vi "MainVI_v1.vi"() -> ()   [LabVIEW 2019]
uses:
  ModBusValue.ctl
  <vilib>/numeric/Random Number (Range) U64.vi
  <vilib>/numeric/sub_Random U32.vi
panel:
  out "문자열[]":string[](array[string])
  in  "아이템 이름":string[][](array[string])=[["1", "Pick&Place Robot", "산업용로봇", "두산로보틱스", "M1509", "ModBusTCP/IP", "192.168.0.100", "200", "대기"], ["2", "", "", "", "", "", "", "", ""], ["3", "", "", "", "", "", "", "", ""], ["4", "", "", "", "", "", "", "", ""], ["5", "", "", "", "", "", "", "", ""], ["6", "", "", "", "", "", "", "", ""], ["7", "", "", "", "", "", "", "", ""], ["8", "", "", "", "", "", "", "", ""], ["9", "", "", "", "", "", "", "", ""], ["10", "", "", "", "", "", "", "", ""], ["11", "", "", "", "", "", "", "", ""]]
  out "Temperature(cobot)":T1
  out "날짜/시간 문자열":string
  out "SystemDataCluster":T2={"문자열 42"="연결", "문자열 43"="연결", "문자열 44"="끊김", "문자열 45"="끊김", "문자열 46"="끊김", "문자열 47"="끊김", "문자열 48"="끊김", "문자열 49"="끊김"} caption="클러스터"
  in  "MAIN Tab":T3(tab)
  out "Cobot_State":string="정지"
  in  "여러 열 리스트박스 4":i32(listbox)
  out "품질률":u8(slide) scale=0.0..100.0
  out "성능률":u8(slide) scale=0.0..100.0
  out "가동률":u8(slide) scale=0.0..100.0
  out "사이클 횟수 그래프":u8(slide) scale=0.0..100.0
  out "웨이브폼 차트 3":u64(graph)=86
  out "AGV_Battery":u8(slide) scale=0.0..100.0
  out "AGV_Coord":string="팔레타이징"
  out "AGV_Action":string="주행 중"
  out "AGV_Velo":string="0.0m"
  out "AGV_UpTime":string="0h00m"
  in  "AGV 통신 리셋":bool
  in  "AGV 통신 정지":bool
  in  "AGV 통신 시작":bool
  out "AGV_State":string="경고"
  out "웨이브폼 차트 2":u64(graph)=86
  out "숫자형 6":dbl
  out "숫자형 7":dbl
  out "숫자형 8":dbl
  out "숫자형 9":dbl
  out "숫자형 5":dbl
  out "숫자형 4":dbl
  out "숫자형 3":dbl
  out "슬라이드 9":u8(slide) scale=0.0..100.0
  out "슬라이드 8":u8(slide) scale=0.0..100.0
  out "슬라이드 7":u8(slide) scale=0.0..100.0
  out "슬라이드 6":u8(slide) scale=0.0..100.0
  out "슬라이드 5":u8(slide) scale=0.0..100.0
  out "슬라이드 4":u8(slide) scale=0.0..100.0
  out "슬라이드 3":u8(slide) scale=0.0..100.0
  out "Cobot_Servo":string="서보 OFF"
  out "Cobot_Task":string="STOP"
  out "Cobot_Cycle":string="0"
  out "Cobot_Comple":string="0/200"
  out "Cobot_UpTime":string="0h00m"
  in  "협동로봇 통신 시작":bool
  in  "협동로봇 통신 리셋":bool
  in  "협동로봇 통신 정지":bool
  out "AMR_Battery":u8(slide) scale=0.0..100.0
  out "AMR_Coord":string="충전스테이션"
  out "AMR_Action":string="주행 중"
  out "AMR_Velo":string="0.0m/s"
  out "AMR_UpTime":string="0h00m"
  in  "AMR 통신 리셋":bool
  in  "AMR 통신 정지":bool
  in  "AMR 통신 시작":bool
  out "AMR_State":string="운전"
  out "Delta_Task":string="자동 검사"
  out "Delta_Cycle":string="0"
  out "Delta_Defective":string="0"
  out "Delta_UpTime":string="0h00m"
  out "Delta_Accuracy":u8(slide) scale=0.0..100.0
  out "IndustRobot_1_Servo":string="서보 OFF"
  out "IndustRobot_1_Task":string="자동 운전"
  out "IndustRobot_1_Cycle":string="100"
  out "IndusRobot_1_Comple":string
  out "IndustRobot_1_UpTime":string="0h00m"
  out "IndustRobot_2_Servo":string="서보 OFF"
  out "IndustRobot_2_Task":string="STOP"
  out "IndustRobot_2_Cycle":string="0"
  out "IndustRobot_2_Comple":string="0"
  out "IndustRobot_2_UpTime":string="0h00m"
  out "IndustRobot_3_Servo":string="서보 OFF"
  out "IndustRobot_3_Task":string="비상 정지"
  out "IndustRobot_3_Cycle":string="0"
  out "IndustRobot_3_Comple":string="0"
  out "IndustRobot_3_UpTime":string="0h00m"
  in  "델타로봇 통신 시작":bool
  in  "델타로봇 통신 리셋":bool
  in  "델타로봇 통신 정지":bool
  in  "산업용로봇 통신 시작":bool
  in  "산업용로봇 통신 리셋":bool
  in  "산업용로봇 통신 정지":bool
  in  "산업용로봇2 통신 시작":bool
  in  "산업용로봇2 통신 리셋":bool
  in  "산업용로봇2 통신 정지":bool
  in  "산업용로봇3 통신 시작":bool
  in  "산업용로봇3 통신 리셋":bool
  in  "산업용로봇3 통신 정지":bool
  out "Delta_State":string="정지"
  out "IndustRobot_1_State":string="정지"
  out "IndustRobot_2_State":string="정지"
  out "IndustRobot_3_State":string="정지"
  out "생산 추이(실시간)":u64(graph)
  out "웨이브폼 차트":u64(graph)=86
  in  "Robot Monitoring Tab":T4(tab)
  in  "Cobot Position Tab":enum32{"Joint Position", "Task Position"}(tab)
  out "Joint Position Graph(cobot)":T5(graph)
  out "Task Position Graph(cobot)":T5(graph)
  in  "여러 열 리스트박스 2":i32(listbox)
  out "Joint6 current":dbl
  out "Joint6 torque":dbl
  out "Joint6 Temp":u8(slide) scale=0.0..100.0
  out "Joint5 current":dbl
  out "Joint5 torque":dbl
  out "Joint4 Temp":u8(slide) scale=0.0..100.0
  out "Joint4 current":dbl
  out "Joint4 torque":dbl
  out "Joint4 Temp":u8(slide) scale=0.0..100.0
  out "Task External Force(Cobot)":T6(graph)
  out "Joint Torque(cobot)":T7(graph)
  in  "Cobot Current Tab":T8(tab)
  out "Total Current Graph(cobot)":T9(graph)
  out "Joint3 current":dbl
  out "Joint3 torque":dbl
  out "Joint3 Temp":u8(slide) scale=0.0..100.0
  out "Joint2 current":dbl
  out "Joint2 torque":dbl
  out "Joint2 Temp":u8(slide) scale=0.0..100.0
  out "Joint1 current":dbl
  out "Joint1 torque":dbl
  out "Joint1 Temp":u8(slide) scale=0.0..100.0
  out "CobotServoState":string="OFF"
  out "CobotStatus":string="EMERGENCY STOP"
  out "TCP Ext Force [N]":u64(graph)=86
  out "평균 소모 전류량 [mA]":u64(graph)=86
  out "평균 조인트 온도 [℃]":u64(graph)=86
  in  "여러 열 리스트박스 3":i32(listbox)
  in  "탭 컨트롤":T10(tab)
  out "제조사2":string
  out "IP Address(Cobot) 3":string
  out "모델명2":string
  out "평균 사이클 타임 [sec]":u64(graph)=86
  out "시간당 작업 수량 [EA/h]":u64(graph)=86
  out "전력 사용량 [W]":u64(graph)=86
  out "IP Address(Cobot) 2":string
  out "CobotStatus 2":string="EMERGENCY STOP"
  in  "여러 열 리스트박스":i32(listbox)
  in  "2. 장비 상세 설정":enum32{"협동로봇", "추가"}(tab)
  in  "모델명":string="M1509"
  in  "통신주기":string
  in  "IP Address(Cobot)":string
  in  "장비명":string
  in  "장비유형":u16(ring) items=["협동로봇", "산업용로봇", "델타로봇", "이송로봇", "자동화장비"]
  in  "통신방식":u16(ring) items=["ModBusTCP/IP", "Serial Commuication"]
  in  "제조사LIST":u16(ring) items=["기타", "캠틱종합기술원", "현대로보틱스", "두산로보틱스"]
  out "CobotCommuState":T11
  in  "1. 장비 목록 및 통신 설정":i32(listbox)
  in  "설정":bool
  in  "데이터 분석":bool
  in  "작업 및 알람":bool
  in  "장비 모니터링":bool
  in  "로봇 모니터링":bool
  in  "main":bool
  in  "시스템 정지":bool
  # "시스템 상태"
  # "PLC"
  # "AMR"
  # "AGV"
  # "협동로봇"
  # "산업용로봇1"
  # "산업용로봇2"
  # "산업용로봇3"
  # "델타로봇"
  # "Admin"
  # "관리자"
  # "주요 알람"
  # "테스트 베드 현황"
  # "7. 산업용로봇3"
  # "2. 산업용로봇2"
  # "3. AGR"
  # "1. AMR"
  # "4. 산업용로봇"
  # "5. 델타로봇(비전)"
  # "6. 협동로봇"
  # "로봇  상세 상태"
  # "AGV"
  # "AMR"
  # "협동로봇"
  # "델타로봇(비전)"
  # "산업용로봇"
  # "산업용로봇2"
  # "산업용로봇3"
  # "모터 상태"
  # "%"
  # "모터 상태"
  # "모터 상태"
  # "검사 정확도"
  # "%"
  # "모터 상태"
  # "%"
  # "배터리"
  # "배터리"
  # "현재 작업"
  # "현재 작업"
  # "현재 작업"
  # "현재 작업"
  # "현재 작업"
  # "로봇 위치"
  # "로봇 위치"
  # "사이클 타임"
  # "사이클 타임"
  # "사이클 타임"
  # "검사 수"
  # "현재 작업"
  # "사이클타임"
  # "현재 작업"
  # "완료 수"
  # "완료 수"
  # "완료 수"
  # "불량 수"
  # "완료 수"
  # "이동 속도"
  # "이동 속도"
  # "가동 시간"
  # "가동 시간"
  # "가동 시간"
  # "가동 시간"
  # "가동 시간"
  # "가동 시간"
  # "가동 시간"
  # "Health index"
  # "작업 현황"
  # "AMR"
  # "%"
  # "총 사이클 횟수"
  # "양품 / 불량 수"
  # "설비 종합 효율"
  # "평균 사이클 타임"
  # "설비 가동률"
  # "%"
  # "AGV"
  # "0%"
  # "1,000ea"
  # "양품"
  # "불량"
  # "%"
  # "협동로봇"
  # "500EA"
  # "500EA"
  # "%"
  # "산업용로봇1"
  # "목표"
  # "100EA"
  # "%"
  # "산업용로봇2"
  # "%"
  # "%"
  # "%"
  # "%"
  # "산업용로봇3"
  # "%"
  # "델타로봇"
  # "%"
  # "실시간 KPI"
  # "ROBOT STATUS :"
  # "/   Servo :"
  # "JOINT 1"
  # "℃"
  # "모터 온도"
  # "N/m"
  # "Joint Torque"
  # "mA"
  # "Motor Current"
  # "JOINT 2"
  # "℃"
  # "모터 온도"
  # "N/m"
  # "Joint Torque"
  # "mA"
  # "Motor Current"
  # "JOINT 3"
  # "℃"
  # "모터 온도"
  # "N/m"
  # "Joint Torque"
  # "mA"
  # "Motor Current"
  # "JOINT 4"
  # "℃"
  # "모터 온도"
  # "N/m"
  # "Joint Torque"
  # "mA"
  # "Motor Current"
  # "JOINT 5"
  # "℃"
  # "모터 온도"
  # "Event / Alarm"
  # "N/m"
  # "Joint Torque"
  # "mA"
  # "Motor Current"
  # "JOINT 6"
  # "℃"
  # "모터 온도"
  # "N/m"
  # "Joint Torque"
  # "mA"
  # "Motor Current"
  # "장비 리스트"
  # "장비 위치"
  # "2. 산업용로봇2"
  # "7. 산업용로봇3"
  # "1. AMR"
  # "3. AGR"
  # "4. 산업용로봇"
  # "5. 델타로봇(비전)"
  # "6. 협동로봇"
  # "장비 상세"
  # "장비 알람 / 이벤트"
  # "협동 로봇"
  # "제조사"
  # "총 작업량"
  # "0"
  # "모델 명"
  # "오류 건수"
  # "0"
  # "현재 작업"
  # "Pick & Place"
  # "IP 주소"
  # "사이클 타임"
  # "0.0sec"
  # "위치"
  # "라인A"
  # "가동 시간"
  # "0h 00m"
  # "제어 방식"
  # "장비명"
  # "장비 유형"
  # "제조사"
  # "모델명"
  # "통신 방식"
  # "IP주소"
  # "통신 주기(ms)"
  # "통신상태"
  # "Physical AI Test-Bed Monitoring System"
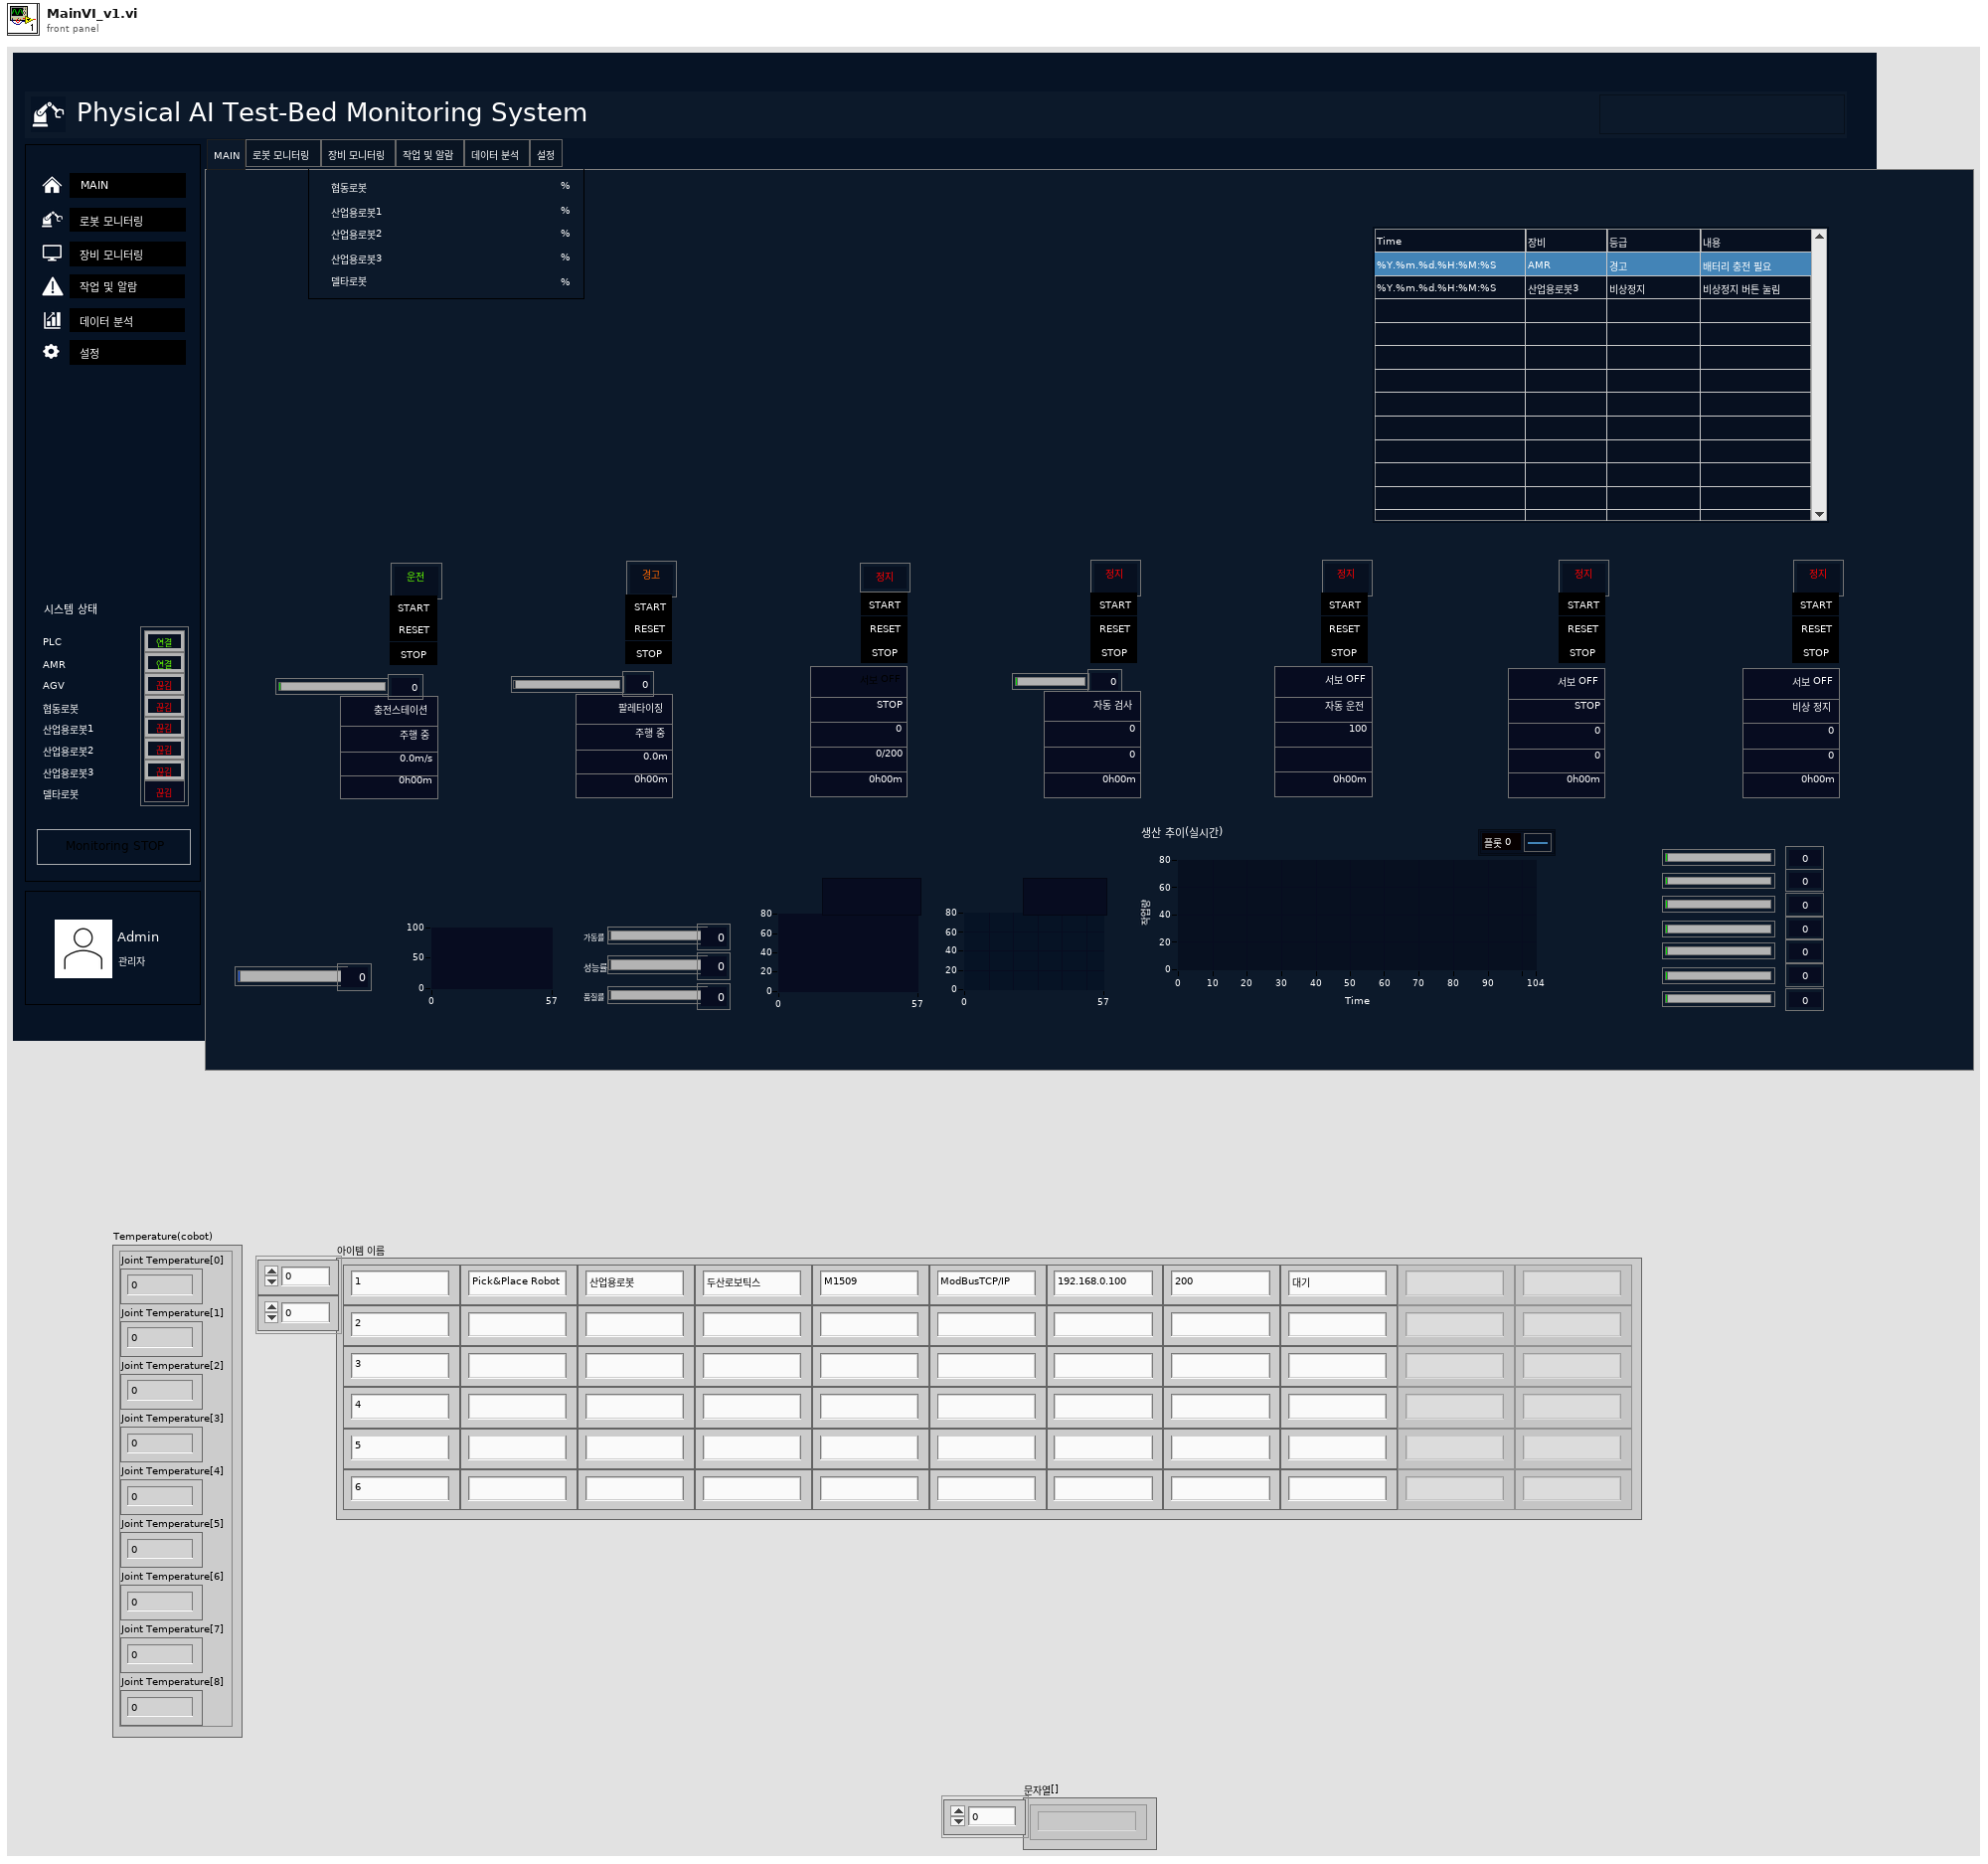
[diagram p1: front panel]
types:
  T1 = cluster{"Joint Temperature[0]":dbl, "Joint Temperature[1]":dbl, "Joint Temperature[2]":dbl, "Joint Temperature[3]":dbl, "Joint Temperature[4]":dbl, "Joint Temperature[5]":dbl, "Joint Temperature[6]":dbl, "Joint Temperature[7]":dbl, "Joint Temperature[8]":dbl}
  T2 = cluster{"문자열 42":string, "문자열 43":string, "문자열 44":string, "문자열 45":string, "문자열 46":string, "문자열 47":string, "문자열 48":string, "문자열 49":string}
  T3 = enum32{"MAIN", "로봇 모니터링", "장비 모니터링", "작업 및 알람", "데이터 분석", "설정"}
  T4 = enum32{"협동로봇", "산업용로봇 1", "산업용로봇 2", "산업용로봇 3", "이송로봇 1", "이송로봇 2"}
  T5 = cluster{"Joint Poistion[0]":dbl, "Joint Poistion[1]":dbl, "Joint Poistion[2]":dbl, "Joint Poistion[3]":dbl, "Joint Poistion[4]":dbl, "Joint Poistion[5]":dbl, "Joint Poistion[6]":dbl, "Joint Poistion[7]":dbl, "Joint Poistion[8]":dbl}
  T6 = cluster{"Joint Torque[0]":dbl, "Joint Torque[1]":dbl, "Joint Torque[2]":dbl, "Joint Torque[3]":dbl, "Joint Torque[4]":dbl, "Joint Torque[5]":dbl, "Joint Torque[6]":dbl, "Joint Torque[7]":dbl, "Joint Torque[8]":dbl}
  T7 = cluster{"External Force[0]":dbl, "External Force[1]":dbl, "External Force[2]":dbl, "External Force[3]":dbl, "External Force[4]":dbl, "External Force[5]":dbl, "External Force[6]":dbl, "External Force[7]":dbl, "External Force[8]":dbl}
  T8 = enum32{"Total", "Joint 1", "Joint 2", "Joint 3", "Joint 4", "Joint 5", "Joint 6"}
  T9 = cluster{"Joint Current[0]":dbl, "Joint Current[1]":dbl, "Joint Current[2]":dbl, "Joint Current[3]":dbl, "Joint Current[4]":dbl, "Joint Current[5]":dbl, "Joint Current[6]":dbl, "Joint Current[7]":dbl, "Joint Current[8]":dbl}
  T10 = enum32{"협동로봇", "산업용로봇 1", "산업용로봇 2", "산업용로봇 3", "델타로봇", "이송로봇 1", "이송로봇 2", "컨베이어 벨트 1", "컨베이어 벨트 2"}
  T11 = typedef "ModBusValue.ctl" = enum16{"대기", "초기화", "읽기", "정지"}
  T12 = cluster{"Joint Poistion[0]":dbl, "Joint Poistion[1]":dbl, "Joint Poistion[2]":dbl, "Joint Poistion[3]":dbl, "Joint Poistion[4]":dbl, "Joint Poistion[5]":dbl, "Joint Poistion[6]":dbl, "Joint Poistion[7]":dbl, "Joint Poistion[8]":dbl}[]
  T13 = enum32{"MAIN", "로봇 모니터링", "장비 모니터링", "작업 및 알람", "데이터 분석", "설정"}[]
  T14 = cluster{"Task Position[0]":dbl, "Task Position[1]":dbl, "Task Position[2]":dbl, "Task Position[3]":dbl, "Task Position[4]":dbl, "Task Position[5]":dbl, "Task Position[6]":dbl, "Task Position[7]":dbl, "Task Position[8]":dbl}
  T15 = cluster{"Robot State[0]":u16, "Robot State[1]":u16, "Robot State[2]":u16, "Robot State[3]":u16, "Robot State[4]":u16, "Robot State[5]":u16, "Robot State[6]":u16, "Robot State[7]":u16, "Robot State[8]":u16}
  T16 = cluster{"TempColorArr[0]":u32, "TempColorArr[1]":u32, "TempColorArr[2]":u32, "TempColorArr[3]":u32, "TempColorArr[4]":u32, "TempColorArr[5]":u32, "TempColorArr[6]":u32, "TempColorArr[7]":u32, "TempColorArr[8]":u32}
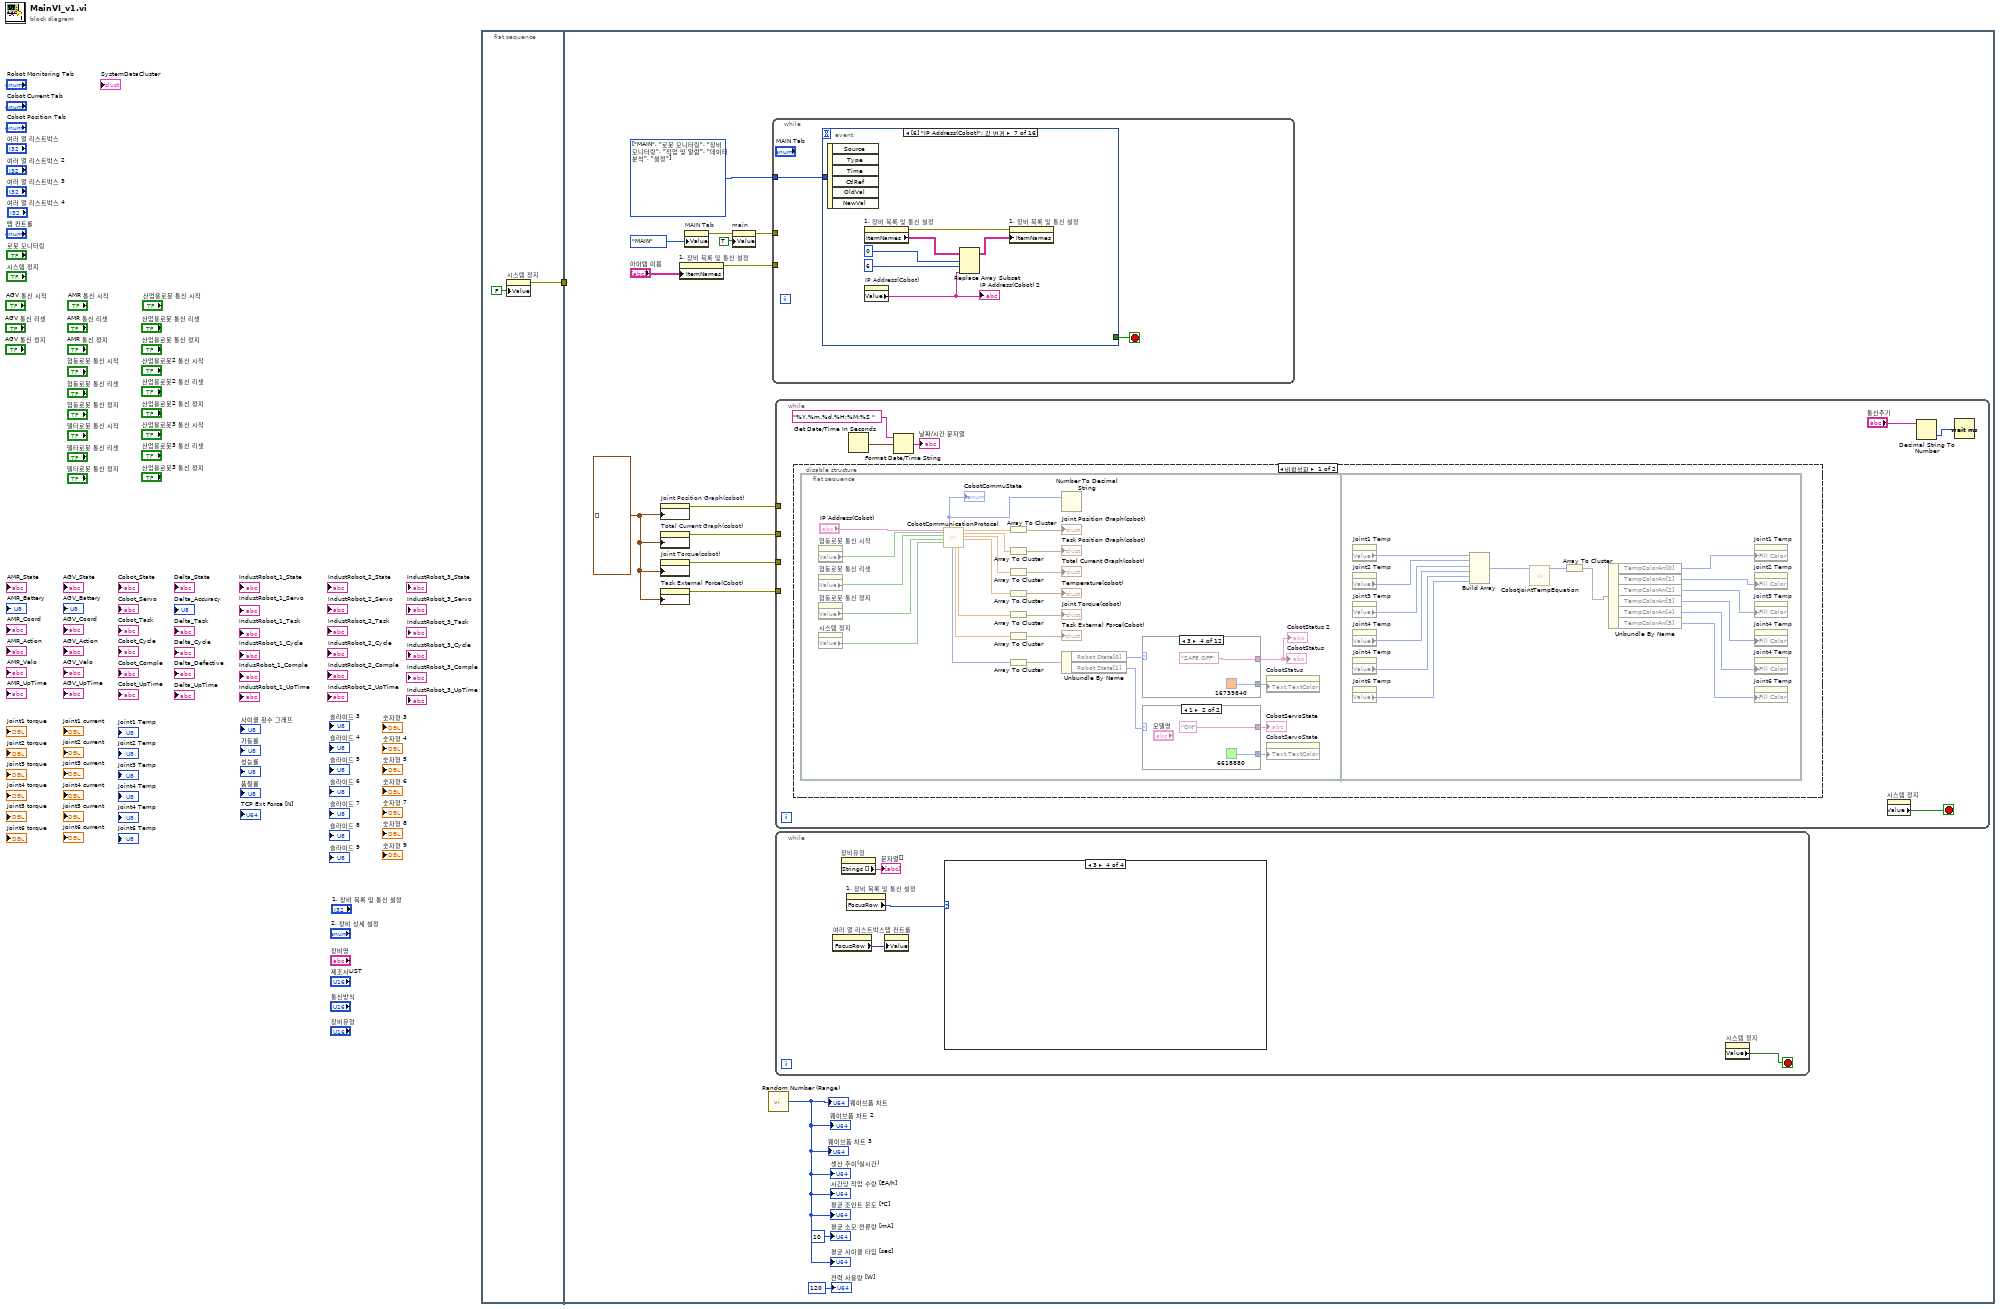
[diagram p0: block diagram]
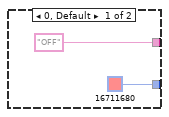
[diagram p5: hidden frame]
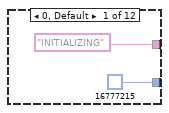
[diagram p6: hidden frame]
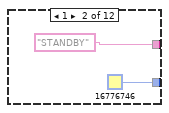
[diagram p7: hidden frame]
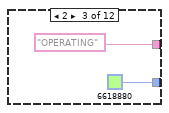
[diagram p8: hidden frame]
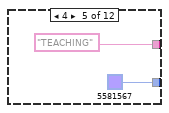
[diagram p9: hidden frame]
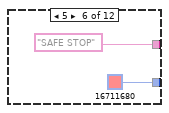
[diagram p10: hidden frame]
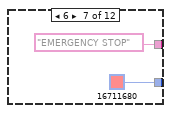
[diagram p11: hidden frame]
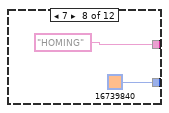
[diagram p12: hidden frame]
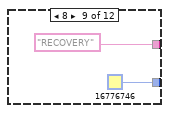
[diagram p13: hidden frame]
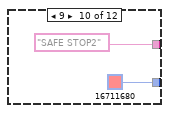
[diagram p14: hidden frame]
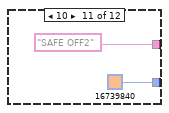
[diagram p15: hidden frame]
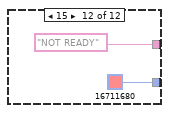
[diagram p16: hidden frame]
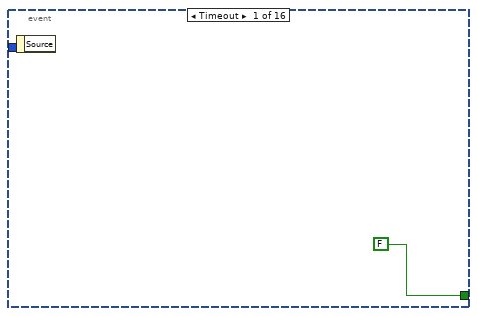
[diagram p18: hidden frame]
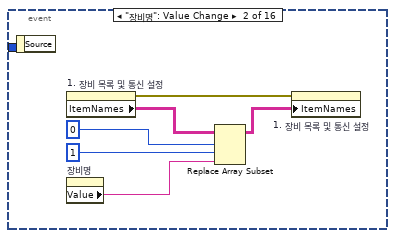
[diagram p19: hidden frame]
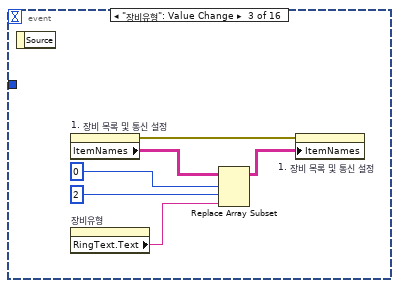
[diagram p20: hidden frame]
diagram:
  n1 = flat-sequence {
    tunnel: [w2] -> w1
    tunnel: w1 -> [_]
    frame #0 {
      n2 = property on="시스템 정지" class="Bool (엄격한)"("Value"=FALSE ("시스템 정지")) -> (error out=w2:errorcluster)  [unwired: 2 in, 1 out]
    }
    frame #1 {
      w13 = T12 [] ("히스토리 데이터")
      w17 = T13 [enum."MAIN", enum."로봇 모니터링", enum."장비 모니터링", enum."작업 및 알람", enum."데이터 분석", enum."설정"] items=["MAIN", "로봇 모니터링", "장비 모니터링", "작업 및 알람", "데이터 분석", "설정"]
      n3 = property on="Joint Position Graph(cobot)" class="WFChart (엄격한)"("History Data"=w13) -> (error out=w12:errorcluster)  [unwired: 2 in, 1 out]
      n4 = property on="Total Current Graph(cobot)" class="WFChart (엄격한)"("History Data"=w13) -> (error out=w11:errorcluster)  [unwired: 2 in, 1 out]
      n5 = property on="Joint Torque(cobot)" class="WFChart (엄격한)"("History Data"=w13) -> (error out=w10:errorcluster)  [unwired: 2 in, 1 out]
      n6 = property on="Task External Force(Cobot)" class="WFChart (엄격한)"("History Data"=w13) -> (error out=w9:errorcluster)  [unwired: 2 in, 1 out]
      n7 = property on="1. 장비 목록 및 통신 설정" class="MCListbox (엄격한)"("ItemNames"="아이템 이름") -> (error out=w4:errorcluster)  [unwired: 2 in, 1 out]
      n8 = property on="MAIN Tab" class="TabCtl (엄격한)"("Value"=T3."MAIN" ("탭 컨트롤")) -> (error out=w15:errorcluster)  [unwired: 2 in, 1 out]
      n9 = property on="main" class="Bool (엄격한)"(error in=w15, "Value"=TRUE ("main")) -> (error out=w16:errorcluster)  [unwired: 1 in, 1 out]
      n10 = call-poly <vilib>:"Random Number (Range).vi"() -> ("number"=→"웨이브폼 차트" →"웨이브폼 차트 2" →"웨이브폼 차트 3" →"생산 추이(실시간)" →"평균 조인트 온도 [℃]" →"평균 사이클 타임 [sec]" →"시간당 작업 수량 [EA/h]":u64)  [unwired: 11 in]
      n11 = while {
        tunnel: w17 -> [w99]
        tunnel: w16 -> [_]
        tunnel: w4 -> [_]
        stop <- w98 stop-if-true
        n12 = event shown="[6] \"IP Address(Cobot)\": 값 변경" {
          selector: _ -> [_ _ _ _ _ _ _ _ _ _ _ _ _ _ _ _]
          dyn-events: _ -> [_ _ _ _ _ _ _ _ _ _ _ _ _ _ _ _]
          timeout: _ -> [_ _ _ _ _ _ _ _ _ _ _ _ _ _ _ _]
          tunnel: w99 -> [_ _ _ _ _ _ _ _ _ w153 w158 w163 w168 w173 w177 _]
          tunnel: [FALSE _ _ _ _ _ _ _ _ FALSE FALSE FALSE FALSE FALSE FALSE TRUE] -> w98
          event Timeout {
            n13 = event-data() -> ()  [unwired: 1 in, 1 out]
          }
          event "장비명": Value Change {
            n14 = event-data() -> ()  [unwired: 1 in, 1 out]
            n15 = property on="1. 장비 목록 및 통신 설정" class="MCListbox (엄격한)"() -> (error out=w104:errorcluster, "ItemNames"=w105:string[][])  [unwired: 2 in, 1 out]
            n16 = property on="장비명" class="Str"() -> ("Value"=w101:string)  [unwired: 2 in, 2 out]
            n17 = Replace Array Subset(array=w105, new element=w101, index (row)=0 ("인덱스 (행)"), index (col)=1 ("비활성화된 인덱스 (열)")) -> (w106:string[][])
            n18 = property on="1. 장비 목록 및 통신 설정" class="MCListbox (엄격한)"(error in=w104, "ItemNames"=w106) -> ()  [unwired: 1 in, 2 out]
          }
          event "장비유형": Value Change {
            n19 = event-data() -> ()  [unwired: 1 in, 1 out]
            n20 = property on="1. 장비 목록 및 통신 설정" class="MCListbox (엄격한)"() -> (error out=w110:errorcluster, "ItemNames"=w111:string[][])  [unwired: 2 in, 1 out]
            n21 = property on="장비유형" class="Ring (엄격한)"() -> ("RingText.Text"=w107:string)  [unwired: 2 in, 2 out]
            n22 = Replace Array Subset(array=w111, new element=w107, index (row)=0 ("인덱스 (행)"), index (col)=2 ("비활성화된 인덱스 (열)")) -> (w112:string[][])
            n23 = property on="1. 장비 목록 및 통신 설정" class="MCListbox (엄격한)"(error in=w110, "ItemNames"=w112) -> ()  [unwired: 1 in, 2 out]
          }
          event "제조사LIST": Value Change {
            n24 = event-data() -> ()  [unwired: 1 in, 1 out]
            n25 = property on="1. 장비 목록 및 통신 설정" class="MCListbox (엄격한)"() -> (error out=w116:errorcluster, "ItemNames"=w117:string[][])  [unwired: 2 in, 1 out]
            n26 = property on="제조사LIST" class="Ring (엄격한)"() -> ("RingText.Text"=w113:string)  [unwired: 2 in, 2 out]
            "제조사2" <- w113
            n27 = Replace Array Subset(array=w117, new element=w113, index (row)=0 ("인덱스 (행)"), index (col)=3 ("비활성화된 인덱스 (열)")) -> (w118:string[][])
            n28 = property on="1. 장비 목록 및 통신 설정" class="MCListbox (엄격한)"(error in=w116, "ItemNames"=w118) -> ()  [unwired: 1 in, 2 out]
          }
          event "모델명": Value Change {
            n29 = event-data() -> ()  [unwired: 1 in, 6 out]
            n30 = property on="모델명" class="Str"() -> ("Value"=w119:string)  [unwired: 2 in, 2 out]
            "모델명2" <- w119
            n31 = property on="1. 장비 목록 및 통신 설정" class="MCListbox (엄격한)"() -> (error out=w122:errorcluster, "ItemNames"=w123:string[][])  [unwired: 2 in, 1 out]
            n32 = Replace Array Subset(array=w123, new element=w119, index (row)=0 ("인덱스 (행)"), index (col)=4 ("비활성화된 인덱스 (열)")) -> (w124:string[][])
            n33 = property on="1. 장비 목록 및 통신 설정" class="MCListbox (엄격한)"(error in=w122, "ItemNames"=w124) -> ()  [unwired: 1 in, 2 out]
          }
          event "통신방식": Value Change {
            n34 = event-data() -> ()  [unwired: 1 in, 6 out]
            n35 = property on="1. 장비 목록 및 통신 설정" class="MCListbox (엄격한)"() -> (error out=w128:errorcluster, "ItemNames"=w129:string[][])  [unwired: 2 in, 1 out]
            n36 = property on="통신방식" class="Ring (엄격한)"() -> ("RingText.Text"=w125:string)  [unwired: 2 in, 2 out]
            "IP Address(Cobot) 3" <- w125
            n37 = Replace Array Subset(array=w129, new element=w125, index (row)=0 ("인덱스 (행)"), index (col)=5 ("비활성화된 인덱스 (열)")) -> (w130:string[][])
            n38 = property on="1. 장비 목록 및 통신 설정" class="MCListbox (엄격한)"(error in=w128, "ItemNames"=w130) -> ()  [unwired: 1 in, 2 out]
          }
          event "IP Address(Cobot)": Value Change {
            n39 = event-data() -> ()  [unwired: 1 in, 6 out]
            n40 = property on="1. 장비 목록 및 통신 설정" class="MCListbox (엄격한)"() -> (error out=w134:errorcluster, "ItemNames"=w135:string[][])  [unwired: 2 in, 1 out]
            n41 = property on="IP Address(Cobot)" class="Str"() -> ("Value"=w131:string)  [unwired: 2 in, 2 out]
            "IP Address(Cobot) 2" <- w131
            n42 = Replace Array Subset(array=w135, new element=w131, index (row)=0 ("인덱스 (행)"), index (col)=6 ("비활성화된 인덱스 (열)")) -> (w136:string[][])
            n43 = property on="1. 장비 목록 및 통신 설정" class="MCListbox (엄격한)"(error in=w134, "ItemNames"=w136) -> ()  [unwired: 1 in, 2 out]
          }
          event "통신주기": Value Change {
            n44 = event-data() -> ()  [unwired: 1 in, 6 out]
            n45 = property on="1. 장비 목록 및 통신 설정" class="MCListbox (엄격한)"() -> (error out=w140:errorcluster, "ItemNames"=w141:string[][])  [unwired: 2 in, 1 out]
            n46 = property on="통신주기" class="Str"() -> ("Value"=w137:string)  [unwired: 2 in, 2 out]
            n47 = Replace Array Subset(array=w141, new element=w137, index (row)=0 ("인덱스 (행)"), index (col)=7 ("비활성화된 인덱스 (열)")) -> (w142:string[][])
            n48 = property on="1. 장비 목록 및 통신 설정" class="MCListbox (엄격한)"(error in=w140, "ItemNames"=w142) -> ()  [unwired: 1 in, 2 out]
          }
          event Value Change {
            n49 = event-data() -> ()  [unwired: 1 in, 6 out]
            n50 = property on="1. 장비 목록 및 통신 설정" class="MCListbox (엄격한)"() -> (error out=w146:errorcluster, "ItemNames"=w147:string[][])  [unwired: 2 in, 1 out]
            n51 = property on="CobotCommuState" class="Enum (엄격한)"() -> ("RingText.Text"=w143:string)  [unwired: 2 in, 2 out]
            n52 = Replace Array Subset(array=w147, new element=w143, index (row)=0 ("인덱스 (행)"), index (col)=8 ("비활성화된 인덱스 (열)")) -> (w148:string[][])
            n53 = property on="1. 장비 목록 및 통신 설정" class="MCListbox (엄격한)"(error in=w146, "ItemNames"=w148) -> ()  [unwired: 1 in, 2 out]
          }
          event "main": Value Change {
            w149 = FALSE
            n54 = event-data() -> ()  [unwired: 1 in, 1 out]
            n55 = Index Array(array=w153, index=0 ("인덱스")) -> (element=w152:T3)
            n56 = property on="MAIN Tab" class="TabCtl (엄격한)"("Value"=w152) -> ()  [unwired: 2 in, 2 out]
            n57 = property on="로봇 모니터링" class="Bool (엄격한)"("Value"=w149) -> ()  [unwired: 2 in, 2 out]
            n58 = property on="장비 모니터링" class="Bool (엄격한)"("Value"=w149) -> ()  [unwired: 2 in, 2 out]
            n59 = property on="작업 및 알람" class="Bool (엄격한)"("Value"=w149) -> ()  [unwired: 2 in, 2 out]
            n60 = property on="데이터 분석" class="Bool (엄격한)"("Value"=w149) -> ()  [unwired: 2 in, 2 out]
            n61 = property on="설정" class="Bool (엄격한)"("Value"=w149) -> ()  [unwired: 2 in, 2 out]
          }
          event "로봇 모니터링": Value Change {
            w154 = FALSE ("main")
            n62 = event-data() -> ()  [unwired: 1 in, 1 out]
            n63 = Index Array(array=w158, index=1 ("인덱스")) -> (element=w156:T3)
            n64 = property on="MAIN Tab" class="TabCtl (엄격한)"("Value"=w156) -> ()  [unwired: 2 in, 2 out]
            n65 = property on="main" class="Bool (엄격한)"("Value"=w154) -> ()  [unwired: 2 in, 2 out]
            n66 = property on="장비 모니터링" class="Bool (엄격한)"("Value"=w154) -> ()  [unwired: 2 in, 2 out]
            n67 = property on="작업 및 알람" class="Bool (엄격한)"("Value"=w154) -> ()  [unwired: 2 in, 2 out]
            n68 = property on="데이터 분석" class="Bool (엄격한)"("Value"=w154) -> ()  [unwired: 2 in, 2 out]
            n69 = property on="설정" class="Bool (엄격한)"("Value"=w154) -> ()  [unwired: 2 in, 2 out]
          }
          event "장비 모니터링": Value Change {
            w159 = FALSE
            n70 = event-data() -> ()  [unwired: 1 in, 1 out]
            n71 = Index Array(array=w163, index=2 ("인덱스")) -> (element=w161:T3)
            n72 = property on="MAIN Tab" class="TabCtl (엄격한)"("Value"=w161) -> ()  [unwired: 2 in, 2 out]
            n73 = property on="main" class="Bool (엄격한)"("Value"=w159) -> ()  [unwired: 2 in, 2 out]
            n74 = property on="로봇 모니터링" class="Bool (엄격한)"("Value"=w159) -> ()  [unwired: 2 in, 2 out]
            n75 = property on="작업 및 알람" class="Bool (엄격한)"("Value"=w159) -> ()  [unwired: 2 in, 2 out]
            n76 = property on="데이터 분석" class="Bool (엄격한)"("Value"=w159) -> ()  [unwired: 2 in, 2 out]
            n77 = property on="설정" class="Bool (엄격한)"("Value"=w159) -> ()  [unwired: 2 in, 2 out]
          }
          event "작업 및 알람": Value Change {
            w164 = FALSE
            n78 = event-data() -> ()  [unwired: 1 in, 1 out]
            n79 = Index Array(array=w168, index=3 ("인덱스")) -> (element=w166:T3)
            n80 = property on="MAIN Tab" class="TabCtl (엄격한)"("Value"=w166) -> ()  [unwired: 2 in, 2 out]
            n81 = property on="main" class="Bool (엄격한)"("Value"=w164) -> ()  [unwired: 2 in, 2 out]
            n82 = property on="로봇 모니터링" class="Bool (엄격한)"("Value"=w164) -> ()  [unwired: 2 in, 2 out]
            n83 = property on="장비 모니터링" class="Bool (엄격한)"("Value"=w164) -> ()  [unwired: 2 in, 2 out]
            n84 = property on="데이터 분석" class="Bool (엄격한)"("Value"=w164) -> ()  [unwired: 2 in, 2 out]
            n85 = property on="설정" class="Bool (엄격한)"("Value"=w164) -> ()  [unwired: 2 in, 2 out]
          }
          event "데이터 분석": Value Change {
            w169 = FALSE
            n86 = event-data() -> ()  [unwired: 1 in, 1 out]
            n87 = Index Array(array=w173, index=4 ("인덱스")) -> (element=w171:T3)
            n88 = property on="MAIN Tab" class="TabCtl (엄격한)"("Value"=w171) -> ()  [unwired: 2 in, 2 out]
            n89 = property on="로봇 모니터링" class="Bool (엄격한)"("Value"=w169) -> ()  [unwired: 2 in, 2 out]
            n90 = property on="장비 모니터링" class="Bool (엄격한)"("Value"=w169) -> ()  [unwired: 2 in, 2 out]
            n91 = property on="작업 및 알람" class="Bool (엄격한)"("Value"=w169) -> ()  [unwired: 2 in, 2 out]
            n92 = property on="설정" class="Bool (엄격한)"("Value"=w169) -> ()  [unwired: 2 in, 2 out]
            n93 = property on="main" class="Bool (엄격한)"("Value"=w169) -> ()  [unwired: 2 in, 2 out]
          }
          event "설정": Value Change {
            w174 = FALSE
            n94 = event-data() -> ()  [unwired: 1 in, 1 out]
            n95 = Index Array(array=w177, index=5 ("인덱스")) -> (element=w176:T3)
            n96 = property on="MAIN Tab" class="TabCtl (엄격한)"("Value"=w176) -> ()  [unwired: 2 in, 2 out]
            n97 = property on="로봇 모니터링" class="Bool (엄격한)"("Value"=w174) -> ()  [unwired: 2 in, 2 out]
            n98 = property on="장비 모니터링" class="Bool (엄격한)"("Value"=w174) -> ()  [unwired: 2 in, 2 out]
            n99 = property on="작업 및 알람" class="Bool (엄격한)"("Value"=w174) -> ()  [unwired: 2 in, 2 out]
            n100 = property on="데이터 분석" class="Bool (엄격한)"("Value"=w174) -> ()  [unwired: 2 in, 2 out]
            n101 = property on="main" class="Bool (엄격한)"("Value"=w174) -> ()  [unwired: 2 in, 2 out]
          }
          event "시스템 정지": Value Change {
            w179 = FALSE
            n102 = event-data() -> ()  [unwired: 1 in, 6 out]
            n103 = property on="로봇 모니터링" class="Bool (엄격한)"("Value"=w179) -> ()  [unwired: 2 in, 2 out]
            n104 = property on="장비 모니터링" class="Bool (엄격한)"("Value"=w179) -> ()  [unwired: 2 in, 2 out]
            n105 = property on="작업 및 알람" class="Bool (엄격한)"("Value"=w179) -> ()  [unwired: 2 in, 2 out]
            n106 = property on="데이터 분석" class="Bool (엄격한)"("Value"=w179) -> ()  [unwired: 2 in, 2 out]
            n107 = property on="설정" class="Bool (엄격한)"("Value"=w179) -> ()  [unwired: 2 in, 2 out]
            n108 = property on="main" class="Bool (엄격한)"("Value"=w179) -> ()  [unwired: 2 in, 2 out]
          }
        }
      }
      n109 = while {
        tunnel: w12 -> [_]
        tunnel: w11 -> [_]
        tunnel: w10 -> [_]
        tunnel: w9 -> [_]
        stop <- w28 stop-if-true
        n110 = disable-structure shown="비활성화" {
          frame Disabled {
            n111 = flat-sequence {
              frame #0 {
                n112 = property on="협동로봇 통신 시작" class="Bool (엄격한)"() -> ("Value"=w54:bool)  [unwired: 2 in, 2 out]
                n113 = property on="협동로봇 통신 리셋" class="Bool (엄격한)"() -> ("Value"=w53:bool)  [unwired: 2 in, 2 out]
                n114 = property on="협동로봇 통신 정지" class="Bool (엄격한)"() -> ("Value"=w52:bool)  [unwired: 2 in, 2 out]
                n115 = property on="시스템 정지" class="Bool (엄격한)"() -> ("Value"=w51:bool)  [unwired: 2 in, 2 out]
                n116 = call "CobotCommunicationProtocal.vi"("address"="IP Address(Cobot)", "협동로봇 통신 시작"=w54, "협동로봇 통신 리셋"=w53, "협동로봇 통신 정지"=w52, "정지"=w51) -> ("상태"=w31:T11, "Robot State"=w38:u16[], "Joint Torque"=w41:dbl[], "External Force"=w42:dbl[], "Joint Poistion"=w50:dbl[], "Task Position"=w48:dbl[], "Joint Current"=w47:dbl[], "Joint Temperature"=w46:dbl[])  [unwired: 6 in, 1 out]
                "CobotCommuState" <- w31
                n117 = Array To Cluster(array=w50) -> (cluster=→"Joint Position Graph(cobot)":T5)
                n118 = Array To Cluster(array=w48) -> (cluster=→"Task Position Graph(cobot)":T14)
                n119 = Array To Cluster(array=w47) -> (cluster=→"Total Current Graph(cobot)":T9)
                n120 = Array To Cluster(array=w46) -> (cluster=→"Temperature(cobot)":T1)
                n121 = Array To Cluster(array=w42) -> (cluster=→"Joint Torque(cobot)":T7)
                n122 = Array To Cluster(array=w41) -> (cluster=→"Task External Force(Cobot)":T6)
                n123 = Array To Cluster(array=w38) -> (cluster=w37:T15)
                n124 = Number To Decimal String(number=w31) -> ()  [unwired: 1 in, 1 out]
                n125 = Unbundle By Name(w37) -> ("Robot State[0]"=w36:u16, "Robot State[1]"=w34:u16)
                n126 = case shown="3" w36 {
                  tunnel: ["INITIALIZING" "STANDBY" "OPERATING" "SAFE OFF" "TEACHING" "SAFE STOP" "EMERGENCY STOP" "HOMING" "RECOVERY" "SAFE STOP2" "SAFE OFF2" "NOT READY"] -> w29
                  tunnel: [u32 16777215 u32 16776746 u32 6618880 u32 16739840 u32 5581567 u32 16711680 u32 16711680 u32 16739840 u32 16776746 u32 16711680 u32 16739840 u32 16711680] -> w35
                  frame 0, Default {
                  }
                  frame 1 {
                  }
                  frame 2 {
                  }
                  frame 3 {
                  }
                  frame 4 {
                  }
                  frame 5 {
                  }
                  frame 6 {
                  }
                  frame 7 {
                  }
                  frame 8 {
                  }
                  frame 9 {
                  }
                  frame 10 {
                  }
                  frame 15 {
                  }
                }
                "CobotStatus" <- w29
                "CobotStatus 2" <- w29
                n127 = case shown="1" w34 {
                  tunnel: ["OFF" "ON"] -> w33
                  tunnel: [u32 16711680 u32 6618880] -> w32
                  frame 0, Default {
                  }
                  frame 1 {
                  }
                }
                "CobotServoState" <- w33
                n128 = property on="CobotStatus" class="Str"("Text.TextColor"=w35) -> ()  [unwired: 2 in, 2 out]
                n129 = property on="CobotServoState" class="Str"("Text.TextColor"=w32) -> ()  [unwired: 2 in, 2 out]
              }
              frame #1 {
                n130 = property on="Joint1 Temp" class="Slide (엄격한)"() -> ("Value"=w88:u8)  [unwired: 2 in, 2 out]
                n131 = property on="Joint2 Temp" class="Slide (엄격한)"() -> ("Value"=w90:u8)  [unwired: 2 in, 2 out]
                n132 = property on="Joint3 Temp" class="Slide (엄격한)"() -> ("Value"=w91:u8)  [unwired: 2 in, 2 out]
                n133 = property on="Joint4 Temp" class="Slide (엄격한)"() -> ("Value"=w92:u8)  [unwired: 2 in, 2 out]
                n134 = property on="Joint4 Temp" class="Slide (엄격한)"() -> ("Value"=w93:u8)  [unwired: 2 in, 2 out]
                n135 = property on="Joint6 Temp" class="Slide (엄격한)"() -> ("Value"=w94:u8)  [unwired: 2 in, 2 out]
                n136 = Build Array(w88, w90, w91, w92, w93, w94) -> (w89:u8[])
                n137 = call "CobotJointTempEquation.vi"("CobotJointTempList"=w89) -> ("TempColorArr"=w95:u32[])  [unwired: 9 in, 1 out]
                n138 = Array To Cluster(array=w95) -> (cluster=w96:T16)
                n139 = Unbundle By Name(w96) -> ("TempColorArr[0]"=w97:u32, "TempColorArr[1]"=w87:u32, "TempColorArr[2]"=w86:u32, "TempColorArr[3]"=w85:u32, "TempColorArr[4]"=w84:u32, "TempColorArr[5]"=w83:u32)
                n140 = property on="Joint1 Temp" class="Slide (엄격한)"("Fill Color"=w97) -> ()  [unwired: 2 in, 2 out]
                n141 = property on="Joint2 Temp" class="Slide (엄격한)"("Fill Color"=w87) -> ()  [unwired: 2 in, 2 out]
                n142 = property on="Joint3 Temp" class="Slide (엄격한)"("Fill Color"=w86) -> ()  [unwired: 2 in, 2 out]
                n143 = property on="Joint4 Temp" class="Slide (엄격한)"("Fill Color"=w85) -> ()  [unwired: 2 in, 2 out]
                n144 = property on="Joint4 Temp" class="Slide (엄격한)"("Fill Color"=w84) -> ()  [unwired: 2 in, 2 out]
                n145 = property on="Joint6 Temp" class="Slide (엄격한)"("Fill Color"=w83) -> ()  [unwired: 2 in, 2 out]
              }
            }
          }
          frame Enabled {
          }
        }
        n146 = Get Date/Time In Seconds() -> (seconds since 1Jan1904=w27:timestamp)
        n147 = Format Date/Time String(time format string (%c)="%Y.%m.%d.%H:%M:%S ", seconds (now)=w27) -> (date/time string=→"날짜/시간 문자열":string)  [unwired: 1 in]
        n148 = property on="시스템 정지" class="Bool (엄격한)"() -> ("Value"=w28:bool)  [unwired: 2 in, 2 out]
        n149 = Decimal String To Number(string="통신주기") -> (number=w23:i32)  [unwired: 2 in, 1 out]
        n150 = Wait (ms)(milliseconds to wait=w23) -> ()  [unwired: 1 out]
      }
      n151 = while {
        stop <- w22 stop-if-true
        n152 = property on="여러 열 리스트박스" class="MCListbox (엄격한)"() -> ("FocusRow"=w19:i32)  [unwired: 2 in, 2 out]
        n153 = property on="장비유형" class="Ring (엄격한)"() -> ("Strings []"=→"문자열[]":string[])  [unwired: 2 in, 2 out]
        n154 = property on="1. 장비 목록 및 통신 설정" class="MCListbox (엄격한)"() -> ("FocusRow"=w21:i32)  [unwired: 2 in, 2 out]
        n155 = property on="탭 컨트롤" class="TabCtl (엄격한)"("Value"=w19) -> ()  [unwired: 2 in, 2 out]
        n156 = case shown="3" w21 {
          frame 0, Default {
          }
          frame 1 {
          }
          frame 2 {
          }
          frame 3 {
          }
        }
        n157 = property on="시스템 정지" class="Bool (엄격한)"() -> ("Value"=w22:bool)  [unwired: 2 in, 2 out]
      }
      "평균 소모 전류량 [mA]" <- u64 10 ("평균 소모 전류량(mA)")
      "전력 사용량 [W]" <- u64 120 ("전력 사용량 (W)")
    }
  }
